vi "ActiveObject_QueueQueue_ProcessRepository_EndevoGoop3.vi"(0 "reference in":refnum<class>, 1 "Action(ReadRepository)":T1(ring), 5 "Error In":errorcluster) -> (9 "ProcessViRef":refnum<vi>, 11 "ProcessSyncQueue":refnum<queue>, 13 "FromProcessQueue":refnum<queue>, 14 "reference out":refnum<class>, 15 "ToProcessQueue":refnum<queue>, 17 "ProcessAlreadyStarted":bool, 19 "Error Out":errorcluster)   [LabVIEW 2020]
uses:
  ActiveObject_QueueQueue_Process.ctl
panel:
  # "Use this indicator for sending messages to the Process VI"
  # "These indicators are used by the process VIs"
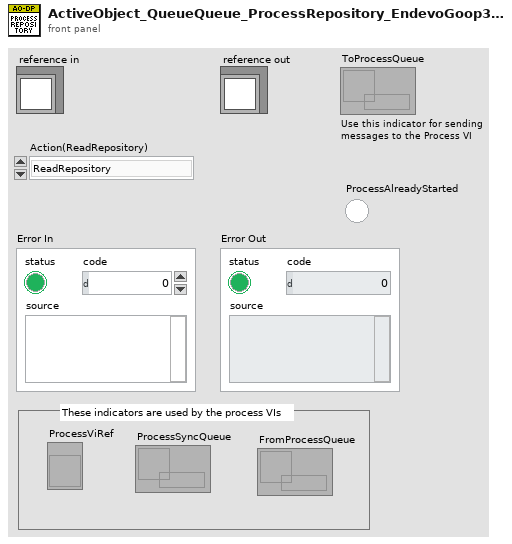
[diagram p1: front panel]
types:
  T1 = enum16{"ReadRepository", "CreateNew", "CreateOrLookUpExisting", "ReadRepositoryAndDestroy"}
  T2 = typedef "ActiveObject_QueueQueue_Process.ctl" = cluster{"ToProcessQueue":refnum<queue>, "FromProcessQueue":refnum<queue>, "ProcessSyncQueue":refnum<queue>, "ProcessViRef":refnum<vi>}
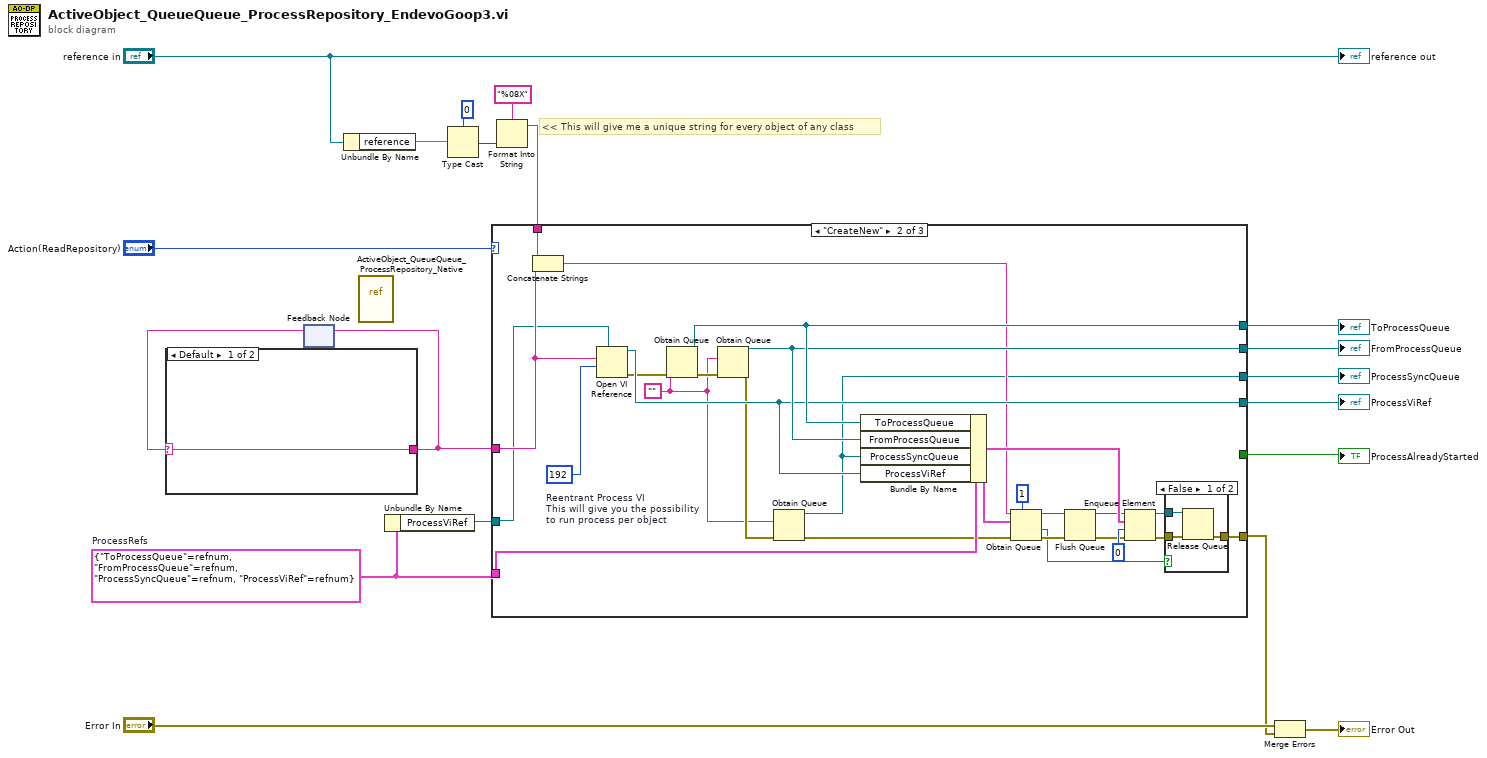
[diagram p0: block diagram]
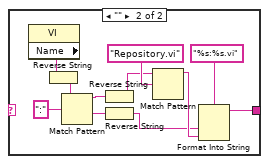
[diagram p2: hidden frame]
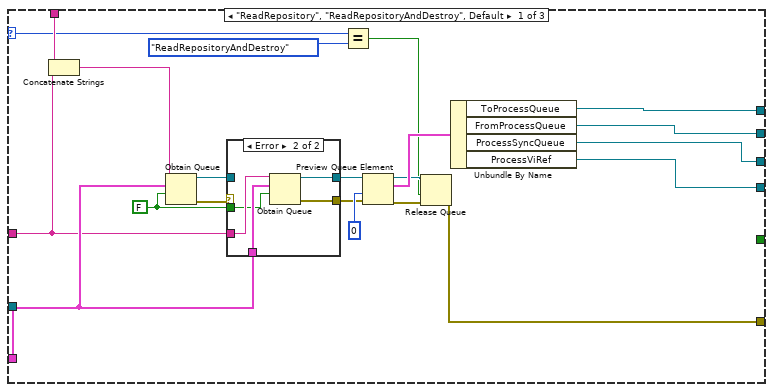
[diagram p3: hidden frame]
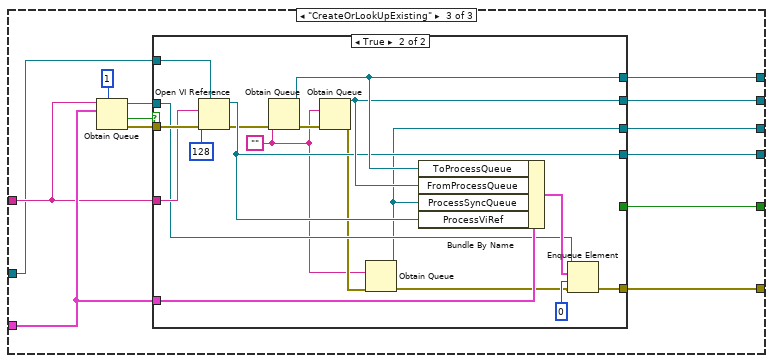
[diagram p6: hidden frame]
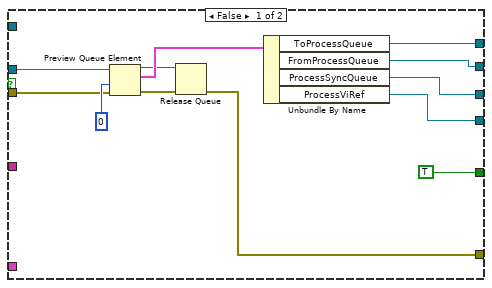
[diagram p7: hidden frame]
diagram:
  w12 = T2 {"ToProcessQueue"=refnum, "FromProcessQueue"=refnum, "ProcessSyncQueue"=refnum, "ProcessViRef"=refnum}  # ProcessRefs
  # "<< This will give me a unique string for every object of any class"
  n1 = feedback #1() -> (w9:string)  [unwired: 1 in]
  n2 = case shown="Default" w9 {
    selector: w9 -> [w20 _]
    tunnel: [w20 w21] -> w10
    frame Default {
    }
    frame "" {
      n3 = property class="VI"() -> ("Name"=w23:string)  [unwired: 2 in, 2 out]
      n4 = Reverse String(1:w23) -> (0:w24:string)
      n5 = Match Pattern(string=w24, regular expression=":") -> (before substring=w28:string, after substring=w25:string)  [unwired: 1 in, 2 out]
      n6 = Reverse String(1:w28) -> (0:w29:string)
      n7 = Reverse String(1:w25) -> (0:w27:string)
      n8 = Match Pattern(string=w29, regular expression="Repository.vi") -> (before substring=w31:string)  [unwired: 1 in, 3 out]
      n9 = Format Into String(format string="%s:%s.vi", w27, w31) -> (resulting string=w21:string)  [unwired: 2 in, 1 out]
    }
  }
  n10 = feedback-in #1(w10) -> ()
  n11 = Unbundle By Name("reference in") -> ("reference"=w14)
  n12 = vi-ref "ActiveObject_QueueQueue_ProcessRepository_Native.vi"() -> ()  [unwired: 1 out]
  n13 = Unbundle By Name(w12) -> ("ProcessViRef"=w11:refnum<vi>)
  n14 = Type Cast(type=u32 0, x=w14) -> (*(type *) &x=w18:u32)
  n15 = Format Into String(format string="%08X", w18) -> (resulting string=w7:string)  [unwired: 2 in, 1 out]
  n16 = case shown="\"CreateNew\"" "Action(ReadRepository)" {
    selector: "Action(ReadRepository)" -> [w34 _ _]
    tunnel: [w47 w68 w100] -> w5
    tunnel: [w49 w85 w102] -> w3
    tunnel: [w48 w84 w101] -> w4
    tunnel: [w50 w83 w99] -> w6
    tunnel: w12 -> [w42 w75 w95]
    tunnel: w7 -> [w40 w74 _]
    tunnel: [w35 w62 w98] -> w1
    tunnel: w10 -> [w39 w72 w91]
    tunnel: [_ _ w93] -> w2
    tunnel: w11 -> [_ w60 w90]
    frame "ReadRepository", "ReadRepositoryAndDestroy", Default {
      w41 = FALSE ("create if not found? (T)")
      n17 = Concatenate Strings(w40, w39) -> (w38:string)
      n18 = Obtain Queue(name (unnamed)=w38, element data type=w42, create if not found? (T)=w41) -> (queue out=w44:refnum<queue>, error out=w46:errorcluster)  [unwired: 2 in, 1 out]
      n19 = case shown="Error" w46 {
        selector: w46 -> [w54 _]
        tunnel: [w54 w56] -> w45
        tunnel: w44 -> [w53 _]
        tunnel: [w53 w57] -> w43
        tunnel: w42 -> [_ w59]
        tunnel: w39 -> [_ w58]
        tunnel: w41 -> [_ w55]
        frame No Error {
        }
        frame Error {
          n20 = Obtain Queue(name (unnamed)=w58, element data type=w59, create if not found? (T)=w55) -> (queue out=w57:refnum<queue>, error out=w56:errorcluster)  [unwired: 2 in, 1 out]
        }
      }
      n21 = Equal?(x=w34, y=T1."ReadRepositoryAndDestroy") -> (x = y?=w33:bool)
      n22 = Preview Queue Element(queue=w43, timeout in ms (-1)=0, error in (no error)=w45) -> (queue out=w37:refnum<queue>, element=w51:T2, error out=w36:errorcluster)  [unwired: 1 out]
      n23 = Release Queue(queue=w37, force destroy? (F)=w33, error in (no error)=w36) -> (error out=w35:errorcluster)  [unwired: 2 out]
      n24 = Unbundle By Name(w51) -> ("ToProcessQueue"=w49:refnum<queue>, "FromProcessQueue"=w48:refnum<queue>, "ProcessSyncQueue"=w47:refnum<queue>, "ProcessViRef"=w50:refnum<vi>)
    }
    frame "CreateNew" {
      w80 = 192  # Reentrant Process VI This will give you the possibility to run process per object
      w69 = ""
      n25 = Concatenate Strings(w74, w72) -> (w73:string)
      n26 = Open VI Reference(type specifier VI Refnum (for type only)=w60, vi path=w72, options=w80) -> (vi reference=w83:refnum<vi>, error out=w81:errorcluster)  [unwired: 3 in]
      n27 = Obtain Queue(element data type=w69, error in (no error)=w81) -> (queue out=w85:refnum<queue>, error out=w82:errorcluster)  [unwired: 3 in, 1 out]
      n28 = Obtain Queue(element data type=w69, error in (no error)=w82) -> (queue out=w84:refnum<queue>, error out=w71:errorcluster)  [unwired: 3 in, 1 out]
      n29 = Obtain Queue(element data type=w69, error in (no error)=w71) -> (queue out=w68:refnum<queue>, error out=w70:errorcluster)  [unwired: 3 in, 1 out]
      n30 = Bundle By Name(cluster=w75, "ToProcessQueue"=w85, "FromProcessQueue"=w84, "ProcessSyncQueue"=w68, "ProcessViRef"=w83) -> (w78:T2)
      n31 = Obtain Queue(max queue size (-1, unlimited)=1, name (unnamed)=w73, element data type=w78, error in (no error)=w70) -> (queue out=w79:refnum<queue>, created new?=w61:bool, error out=w66:errorcluster)  [unwired: 1 in]
      n32 = Flush Queue(queue=w79, error in (no error)=w66) -> (queue out=w67:refnum<queue>, error out=w65:errorcluster)  [unwired: 1 out]
      n33 = Enqueue Element(queue=w67, element=w78, timeout in ms (-1)=0, error in (no error)=w65) -> (queue out=w63:refnum<queue>, error out=w64:errorcluster)  [unwired: 1 out]
      n34 = case shown="False" w61 {
        tunnel: w64 -> [w88 w89]
        tunnel: w63 -> [w87 _]
        tunnel: [w86 w89] -> w62
        frame False {
          n35 = Release Queue(queue=w87, error in (no error)=w88) -> (error out=w86:errorcluster)  [unwired: 1 in, 2 out]
        }
        frame True {
        }
      }
    }
    frame "CreateOrLookUpExisting" {
      n36 = Obtain Queue(max queue size (-1, unlimited)=1, name (unnamed)=w91, element data type=w95) -> (queue out=w96:refnum<queue>, created new?=w97:bool, error out=w94:errorcluster)  [unwired: 2 in]
      n37 = case shown="True" w97 {
        tunnel: [w114 w132] -> w102
        tunnel: [w113 w131] -> w101
        tunnel: [w112 w117] -> w100
        tunnel: [w111 w130] -> w99
        tunnel: [w104 w129] -> w98
        tunnel: w95 -> [_ w128]
        tunnel: w94 -> [w108 w123]
        tunnel: w91 -> [_ w122]
        tunnel: w96 -> [w109 w121]
        tunnel: [TRUE _] -> w93
        tunnel: w90 -> [_ w116]
        frame False {
          n38 = Preview Queue Element(queue=w109, timeout in ms (-1)=0, error in (no error)=w108) -> (queue out=w103:refnum<queue>, element=w107:T2, error out=w105:errorcluster)  [unwired: 1 out]
          n39 = Release Queue(queue=w103, error in (no error)=w105) -> (error out=w104:errorcluster)  [unwired: 1 in, 2 out]
          n40 = Unbundle By Name(w107) -> ("ToProcessQueue"=w114:refnum<queue>, "FromProcessQueue"=w113:refnum<queue>, "ProcessSyncQueue"=w112:refnum<queue>, "ProcessViRef"=w111:refnum<vi>)
        }
        frame True {
          w118 = ""
          n41 = Open VI Reference(type specifier VI Refnum (for type only)=w116, vi path=w122, options=128, error in (no error)=w123) -> (vi reference=w130:refnum<vi>, error out=w126:errorcluster)  [unwired: 2 in]
          n42 = Obtain Queue(element data type=w118, error in (no error)=w126) -> (queue out=w132:refnum<queue>, error out=w127:errorcluster)  [unwired: 3 in, 1 out]
          n43 = Obtain Queue(element data type=w118, error in (no error)=w127) -> (queue out=w131:refnum<queue>, error out=w120:errorcluster)  [unwired: 3 in, 1 out]
          n44 = Obtain Queue(element data type=w118, error in (no error)=w120) -> (queue out=w117:refnum<queue>, error out=w119:errorcluster)  [unwired: 3 in, 1 out]
          n45 = Bundle By Name(cluster=w128, "ToProcessQueue"=w132, "FromProcessQueue"=w131, "ProcessSyncQueue"=w117, "ProcessViRef"=w130) -> (w125:T2)
          n46 = Enqueue Element(queue=w121, element=w125, timeout in ms (-1)=0, error in (no error)=w119) -> (error out=w129:errorcluster)  [unwired: 2 out]
        }
      }
    }
  }
  "ProcessSyncQueue" <- w5
  "ToProcessQueue" <- w3
  "FromProcessQueue" <- w4
  "ProcessViRef" <- w6
  "ProcessAlreadyStarted" <- w2
  n47 = Merge Errors("Error In", w1) -> (→"Error Out":errorcluster)
  "reference out" <- "reference in"
